vi "Channel Interface.vi"(8 "error in (no error)":errorcluster, 11 "Node Ptr":T1 format="%.0x") -> (0 "error out":errorcluster)   [LabVIEW 2020, in "SLSC EDS System Explorer.lvlib"]
uses:
  SLSC EDS System Explorer.lvlib
  <vilib>/NI VeriStand/Custom Device API/Custom Device Item Ref.ctl
  <vilib>/NI VeriStand/Custom Device API/Custom Device Channel Type.ctl
  <vilib>/NI VeriStand/Custom Device Tools/Custom Device Utility Library/Search Direction.ctl
  <vilib>/Utility/miscctls.llb/LVStringsAndValuesArrayTypeDef_U16.ctl
  Shared/Constants.vi
  <vilib>/NI VeriStand/Custom Device API/Get Item Property (String).vi
  <vilib>/NI VeriStand/Custom Device Tools/Custom Device Utility Library/NI VeriStand - Search for Item by GUID.vi
  <vilib>/NI VeriStand/Custom Device API/Custom Device API.lvlib
  Shared/SLSC EDS Shared.lvlib
  <vilib>/NI VeriStand/Custom Device Tools/Custom Device Utility Library/Custom Device Utility Library.lvlib
  SLSC CD API/SLSC CD Shared/SLSC CD Shared.lvlib
  SLSC UI API/SLSC Tree Control.lvlib
  SLSC CD API/SLSC CD System Explorer/SLSC CD System Explorer.lvlib
  <vilib>/NI VeriStand/Custom Device Tools/Custom Device Utility Library/NI VeriStand - Search for Item by Name.vi
panel:
  in  "Property tree":string[](tree)
  out "Physical Channel":string
  out "Property/Command Name":string
  out "Datatype":string
  in  "U8":u8 format="%.0x"
  in  "I8":i8
  in  "U32":u32 format="%.0x"
  in  "I32":i32
  in  "U64":u64 format="%.0x"
  in  "I64":i64
  in  "Ring":u16(ring)
  in  "DBL":dbl format="%#_16g"
  out "Documentation":string
  in  "Default Value":dbl
  out "Access":i32(ring) items=["None", "Read Only", "Write Only", "Read/Write"]
  out "SLSC Debugging Information":string
  in  "Header":cluster{"Section Name":string}={"Section Name"="Custom Device Item Settings"}
  out "Description":string
  out "Name":string
  # "Default Value"
  # "Channel Value"
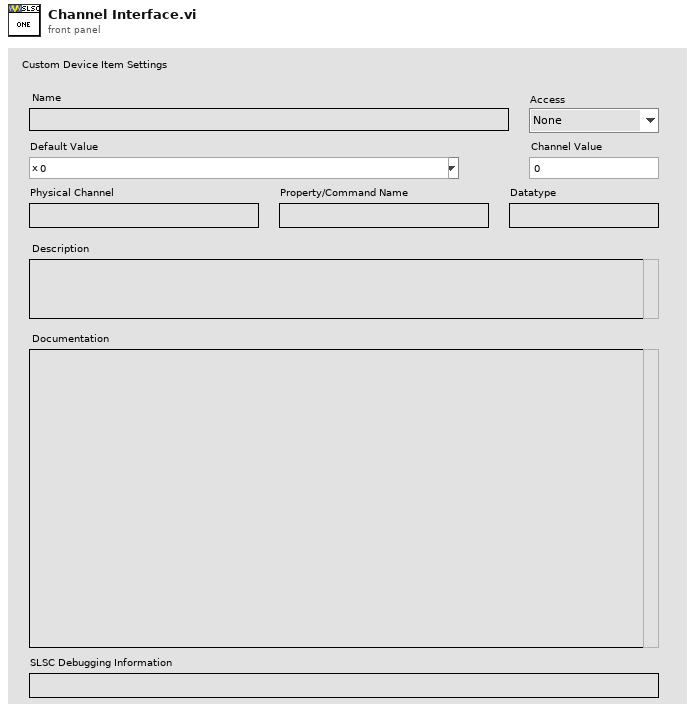
[diagram p1: front panel]
types:
  T1 = typedef "Custom Device API.lvlib/Custom Device Item Ref.ctl" = u64
  T2 = enum8{"Enabled", "Disabled", "Disabled and Grayed Out"}
  T3 = typedef "Custom Device Utility Library.lvlib/Search Direction.ctl" = enum16{"Down", "Up"}
  T4 = typedef "Custom Device API.lvlib/Custom Device Channel Type.ctl" = enum16{"Input", "Output"}
  T5 = typedef "LVStringsAndValuesArrayTypeDef_U16.ctl" = cluster{"String":string, "Value":u16}[]
  T6 = typedef "Custom Device API.lvlib/Custom Device Item Info.ctl" = cluster{"Name":string, "Is Channel":bool, "GUID":string, "Is Waveform":bool}
  T7 = typedef "EDSjsonStructure.ctl" = cluster{"vendorNum":u32, "vendorName":string, "vendorPrefix":string, "productNum":u32, "productName":string, "capsVersion":string, "capsSpecVersion":u32, "capsSpecOldestCompatibleVersion":u32, "enums":T8[], "properties":T9[], "commands":T10[], "scales":T11[], "physicalChannels":T12[], "registerMap":cluster{"registers":T13[]}}
  T8 = typedef "enum.ctl" = cluster{"name":string, "description-en":string, "values":cluster{"name":string, "description-en":string, "value":i32}[]}
  T9 = typedef "property.ctl" = cluster{"name":string, "description-en":string, "documentation-en":string, "dataType":string, "bitfield":string, "access":string, "scale":string, "value":variant, "min":variant, "max":variant, "default value":variant}
  T10 = typedef "command.ctl" = cluster{"name":string, "description-en":string, "documentation-en":string, "startBitfield":string, "waitTimeInMs":i32, "doneBitfield":string, "doneInterrupt":string, "doneTimeoutInMs":i32, "value":variant}
  T11 = typedef "scale.ctl" = cluster{"name":string, "description-en":string, "m":dbl, "b":dbl, "forwardCoeffs":dbl[], "reverseCoeffs":dbl[], "coercion":string, "table":cluster{"scaled":dbl, "unscaled":dbl}[]}
  T12 = typedef "physicalChannel.ctl" = cluster{"name":string, "description-en":string, "commands":T10[], "properties":T9[]}
  T13 = typedef "register.ctl" = cluster{"name":string, "description-en":string, "access":string, "address":u32, "size":u32, "bitfields":cluster{"name":string, "description-en":string, "offset":u32, "size":u32, "signed":bool, "strobe":bool}[]}
  T14 = typedef "Custom Device API.lvlib/Custom Device Channel.ctl" = cluster{"Type":T4, "Units":string, "Default Value":dbl, "Faultable":bool, "Scalable":bool}
  T15 = cluster{"Left Cell String":string, "Child Text":string[], "Child Tag":string, "Item Indent":i32, "Child Only?":bool, "Glyph Index":i32}[]
  T16 = cluster{"Left Cell String":string, "Child Text":string[], "Child Tag":string, "Item Indent":i32, "Child Only?":bool, "Glyph Index":i32}
  T17 = cluster{"name":string, "description-en":string, "value":i32}[]
  T18 = typedef "Custom Device API.lvlib/Custom Device Commands.ctl" = enum16{"Default", "Item renamed", "Shutdown", "Dynamic button pressed"}
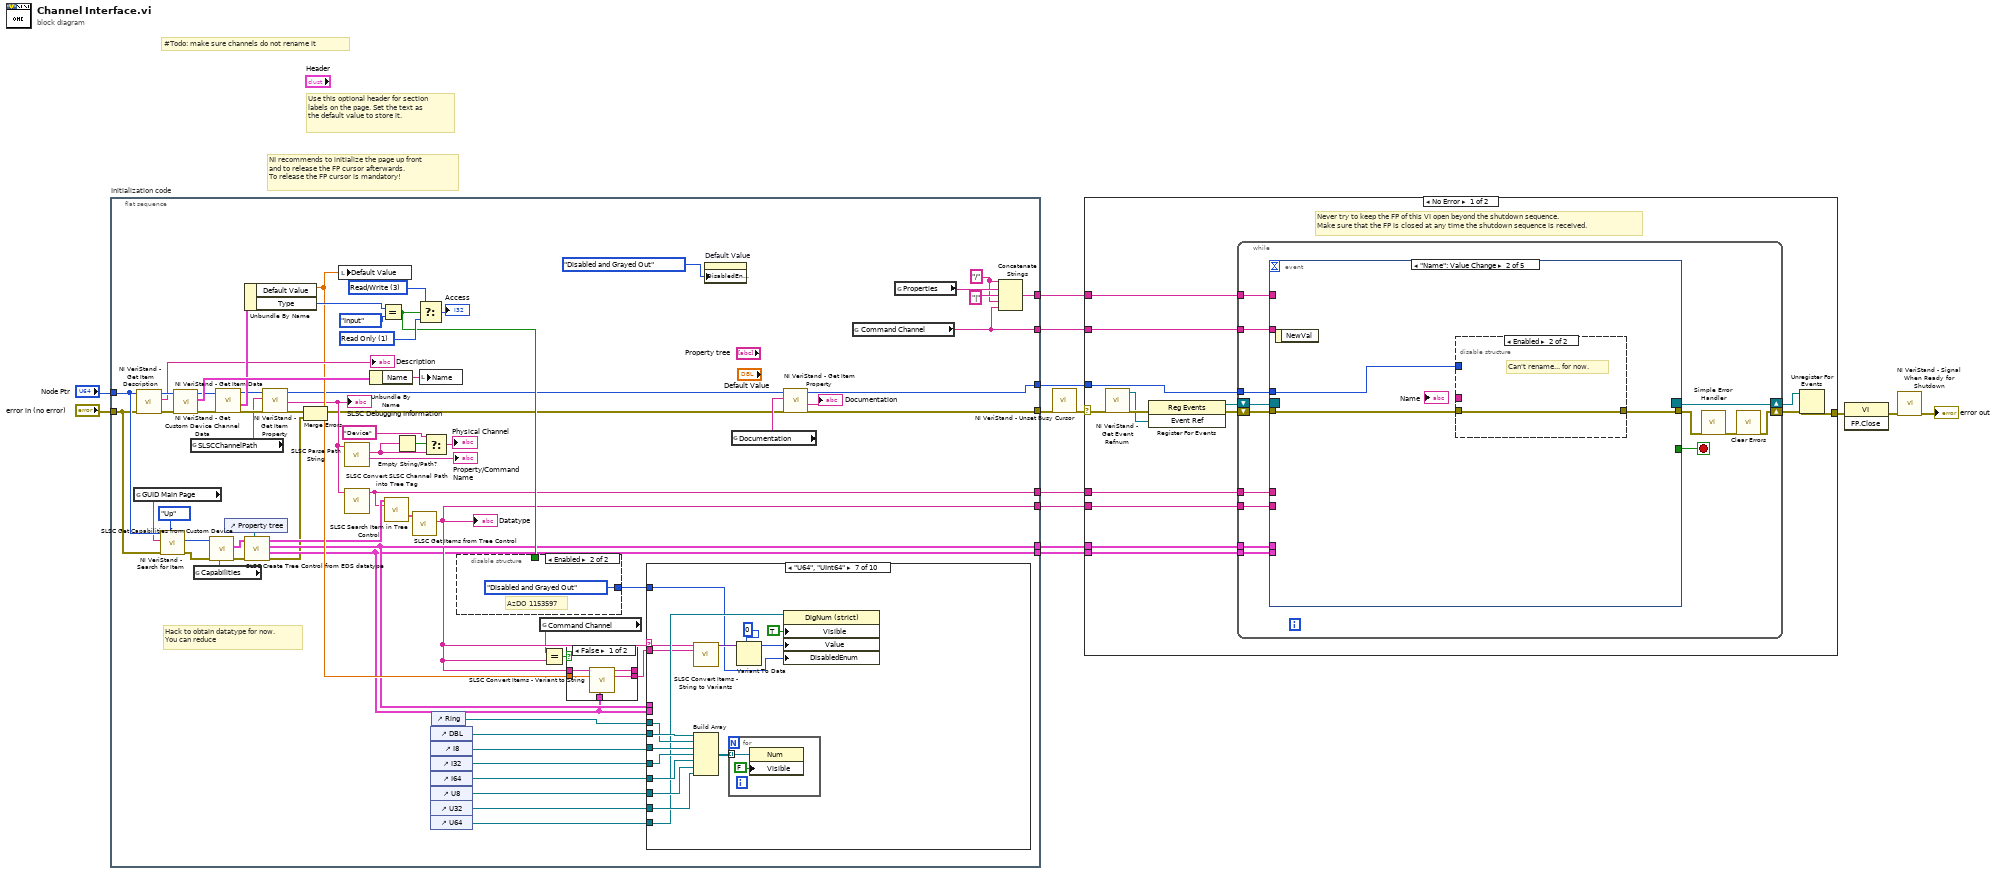
[diagram p0: block diagram]
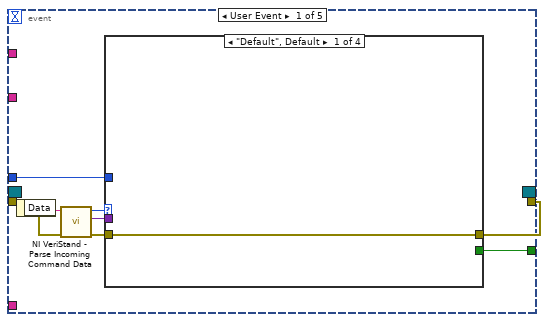
[diagram p2: hidden frame]
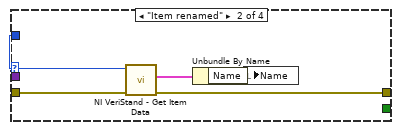
[diagram p3: hidden frame]
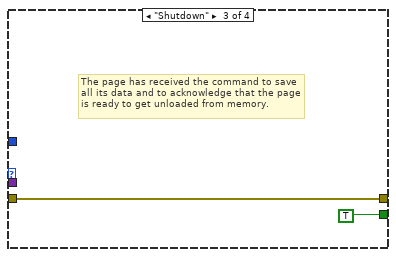
[diagram p4: hidden frame]
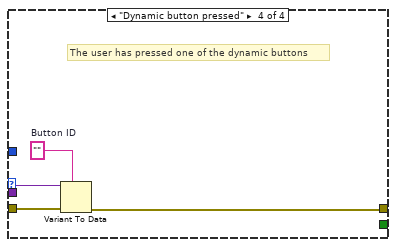
[diagram p5: hidden frame]
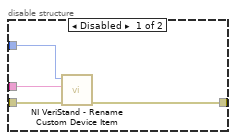
[diagram p6: hidden frame]
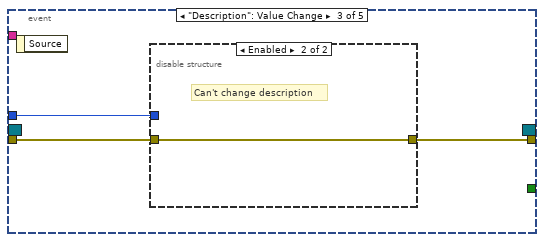
[diagram p7: hidden frame]
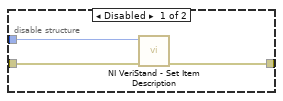
[diagram p8: hidden frame]
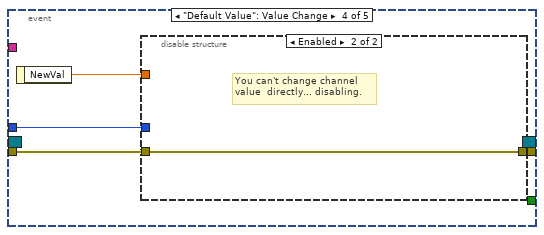
[diagram p9: hidden frame]
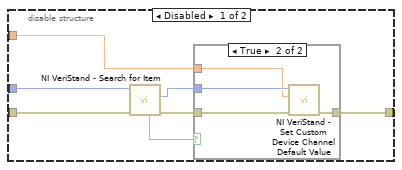
[diagram p10: hidden frame]
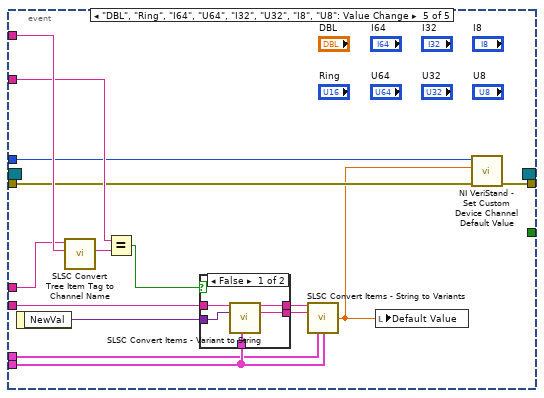
[diagram p12: hidden frame]
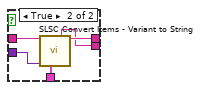
[diagram p13: hidden frame]
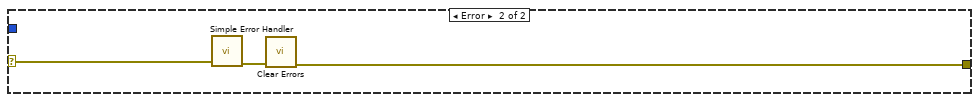
[diagram p14: hidden frame]
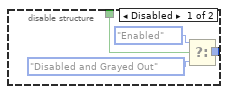
[diagram p15: hidden frame]
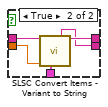
[diagram p16: hidden frame]
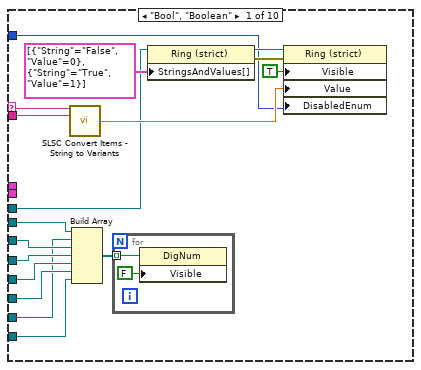
[diagram p17: hidden frame]
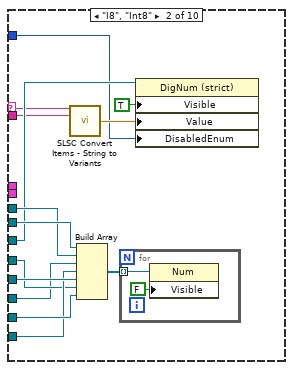
[diagram p18: hidden frame]
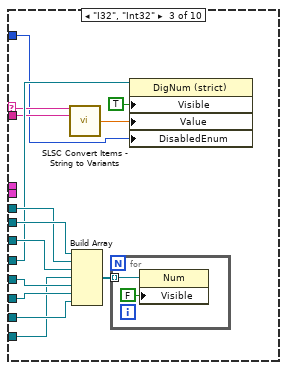
[diagram p19: hidden frame]
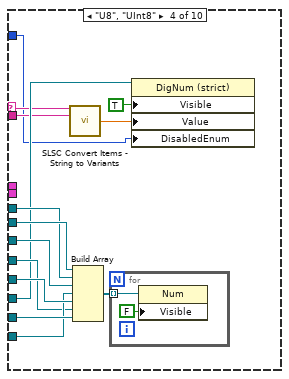
[diagram p20: hidden frame]
diagram:
  # "#Todo: make sure channels do not rename it"
  # "Use this optional header for section labels on the page. Set the text as the default value to store it."
  # "NI recommends to initialize the page up front\nand to release the FP cursor afterwards.\nTo release the FP cursor is mandatory!"
  n1 = flat-sequence "Initialization code" {
    tunnel: "error in (no error)" -> [w27]
    tunnel: "Node Ptr" -> [w52]
    tunnel: [w64] -> w10
    tunnel: [w22] -> w7
    tunnel: [w56] -> w6
    tunnel: [w48] -> w5
    tunnel: [w29] -> w4
    tunnel: [w35] -> w3
    tunnel: [w30] -> w2
    tunnel: [w31] -> w1
    frame #0 {
      w57 = "/" ("string")
      w77 = 1 items=["None", "Read Only", "Write Only", "Read/Write"] ("Access")
      w76 = 3 items=["None", "Read Only", "Write Only", "Read/Write"] ("Access")
      # "Hack to obtain datatype for now.\nYou can reduce"
      n2 = global read "Constants.vi" "GUID Main Page"() -> (w51:string)
      n3 = call <vilib>:"NI VeriStand - Get Item Description.vi"("error in (no error)"=w27, "Item Ref in"=w52) -> ("error out"=w79:errorcluster, "Description"=→"Description":string, "Item Ref out"=w80:T1)  [unwired: 7 out]
      n4 = call-poly <vilib>:"NI VeriStand - Search for Item.vi"("Direction (Down)"=Search_Direction."Up", "error in"=w27, "Item GUID"=w51, "Section Ref in"=w52) -> ("error out"=w28:errorcluster, "Item Ref"=w53:T1)  [unwired: 4 in, 2 out]
      n5 = call <vilib>:"NI VeriStand - Get Item Data.vi"("error in (no error)"=w79, "Item Ref in"=w80) -> ("error out"=w69:errorcluster, "Item Info"=w78:T6, "Item Ref out"=w70:T1)  [unwired: 7 out]
      n6 = global read "Constants.vi" "SLSCChannelPath"() -> (w68:string)
      n7 = global read "Constants.vi" "Capabilities"() -> (w60:string)
      n8 = call "SLSC Get Capabilities from Custom Device.vi"("Property Name"=w60, "error in (no error)"=w28, "Device Item Ref in"=w53) -> ("error out"=w24:errorcluster, "data"=w36:T7)  [unwired: 3 in, 4 out]
      n9 = call <vilib>:"NI VeriStand - Get Custom Device Channel Data.vi"("error in (no error)"=w69, "Channel Ref in"=w70) -> ("error out"=w72:errorcluster, "Channel"=w71:T14, "Channel Ref out"=w66:T1)  [unwired: 4 in, 3 out]
      n10 = control-ref of="Property tree"() -> (w37:refnum<vi>)
      n11 = Unbundle By Name(w71) -> ("Default Value"=w49:dbl, "Type"=w73:T4)
      n12 = call "SLSC Create Tree Control from EDS datatype.vi"("Property Tree"=w37, "error in (no error)"=w24, "SLSC EDS module"=w36) -> ("error out"=w18:errorcluster, "Enum Strings"=w29:cluster{"name":string, string}[], "Enums"=w35:T8[], "SLSC Output Tree"=w34:T15)  [unwired: 5 in]
      n13 = call-poly <vilib>:"NI VeriStand - Get Item Property.vi"("error in (no error)"=w72, "Property Name"=w68, "Item Ref in"=w66) -> ("error out"=w20:errorcluster, "Value"=w33:string, "Item Ref out"=w21:T1)  [unwired: 5 in, 1 out]
      "SLSC Debugging Information" <- w33
      n14 = Merge Errors(w20, w18) -> (w19:errorcluster)
      n15 = local write "Default Value"(w49) -> ()
      n16 = call "SLSC Parse Path String.vi"("SLSC Channel Path"=w33) -> ("Property or Command"=→"Property/Command Name":string, "Physical Channel"=w39:string)  [unwired: 7 in, 2 out]
      n17 = call "SLSC Convert SLSC Channel Path into Tree Tag.vi"("SLSC Channel Path"=w33) -> ("Tree Item Channel"=w31:string)  [unwired: 9 in, 1 out]
      n18 = Unbundle By Name(w78) -> ("Name"=w61:string)
      n19 = Equal?(x=w73, y=Custom_Device_Channel_Type."Input") -> (x = y?=w62:bool)
      n20 = call "SLSC Search Item in Tree Control.vi"("SLSC Output Tree"=w34, "Item Tag"=w31) -> ("Item"=w32:T16)  [unwired: 10 in, 3 out]
      n21 = Empty String/Path?(string/path=w39) -> (empty?=w41:bool)
      n22 = call "SLSC Get Items from Tree Control.vi"("Item"=w32) -> ("Datatype"=w30:string)  [unwired: 6 in, 4 out]
      "Datatype" <- w30
      n23 = Select(t=w76, s=w62, f=w77) -> (s? t:f=→"Access":i32)
      n24 = local write "Name"(w61) -> ()
      n25 = Select(t="Device", s=w41, f=w39) -> (s? t:f=→"Physical Channel":string)
      n26 = control-ref of="DBL"() -> (w43:refnum<vi>)
      n27 = control-ref of="I8"() -> (w55:refnum<vi>)
      n28 = control-ref of="I32"() -> (w54:refnum<vi>)
      n29 = control-ref of="I64"() -> (w44:refnum<vi>)
      n30 = control-ref of="U8"() -> (w47:refnum<vi>)
      n31 = control-ref of="U32"() -> (w46:refnum<vi>)
      n32 = control-ref of="U64"() -> (w45:refnum<vi>)
      n33 = control-ref of="Ring"() -> (w16:refnum<vi>)
      n34 = disable-structure shown="Enabled" {
        disable-tunnel: w62 -> [w84 _]
        disable-tunnel: [w81 T2."Disabled and Grayed Out" ("Disabled")] -> w15
        frame Disabled {
          n35 = Select(t=T2."Enabled" ("Disabled"), s=w84, f=T2."Disabled and Grayed Out" ("Disabled")) -> (s? t:f=w81:T2)
        }
        frame Enabled {
          # "AzDO 1153597"
        }
      }
      n36 = global read "Constants.vi" "Command Channel"() -> (w23:string)
      n37 = Equal?(x=w23, y=w30) -> (x = y?=w26:bool)
      n38 = case shown="False" w26 {
        tunnel: w49 -> [w90 w92]
        tunnel: [w89 w91] -> w25
        tunnel: [w88 w95] -> _
        tunnel: w30 -> [w87 w94]
        tunnel: w29 -> [w86 w93]
        frame False {
          n39 = call "SLSC Convert Items - Variant to String.vi"("Datatype"=w87, "value"=w90, "Enum string"=w86) -> ("Output data type"=w88:string, "string data value"=w89:string)  [unwired: 6 in, 5 out]
        }
        frame True {
          n40 = call "SLSC Convert Items - Variant to String.vi"("Datatype"=w94, "reset value"=w92, "Enum string"=w93) -> ("string data reset value"=w91:string, "Output data type"=w95:string)  [unwired: 6 in, 5 out]
        }
      }
      n41 = case shown="\"U64\", \"UInt64\"" w30 {
        selector: w30 -> [w102 w119 w135 w151 w167 w181 w201 w219 w236 w267]
        tunnel: w16 -> [w98 w127 w143 w159 w174 w193 w211 w228 w232 w259]
        tunnel: w46 -> [w105 w124 w138 w155 w176 w188 w205 w222 w241 w271]
        tunnel: w43 -> [w112 w128 w144 w160 w175 w194 w212 w221 w246 w276]
        tunnel: w55 -> [w111 w120 w142 w158 w173 w192 w210 w227 w245 w275]
        tunnel: w54 -> [w110 w122 w136 w153 w172 w191 w209 w226 w244 w274]
        tunnel: w44 -> [w109 w126 w141 w157 w171 w186 w208 w225 w243 w273]
        tunnel: w47 -> [w108 w121 w140 w152 w170 w190 w207 w224 w242 w272]
        tunnel: w45 -> [w107 w123 w137 w154 w169 w187 w204 w220 w240 w270]
        tunnel: w35 -> [_ _ _ _ _ _ _ _ w247 _]
        tunnel: w25 -> [w101 w118 w134 w150 w166 w180 w200 w218 w238 w268]
        tunnel: w29 -> [_ _ _ _ _ _ _ _ w237 _]
        tunnel: w15 -> [w96 w115 w131 w147 w163 w179 w197 w215 w231 _]
        frame "Bool", "Boolean" {
          n42 = call "SLSC Convert Items - String to Variants.vi"("Datatype"=w102, "Value"=w101) -> ("Value (DBL)"=w100:dbl)  [unwired: 10 in, 3 out]
          n43 = Build Array(w112, w105, w111, w110, w109, w108, w107) -> (w106:refnum<vi>[])
          n44 = for {
            tunnel: w106 -> [w114] mode=indexing
            n45 = property class="DigNum"(reference=w114, "Visible"=FALSE) -> ()  [unwired: 1 in, 2 out]
          }
          n46 = property on="Property Node" class="Ring (strict)"(reference=w98, "StringsAndValues[]"=T5 [{"String"="False", "Value"=0}, {"String"="True", "Value"=1}] ("Strings And Values []")) -> (reference out=w97:refnum<vi>, error out=w103:errorcluster)  [unwired: 1 in]
          n47 = property class="Ring (strict)"(reference=w97, error in=w103, "Visible"=TRUE, "Value"=w100, "DisabledEnum"=w96) -> ()  [unwired: 2 out]
        }
        frame "I8", "Int8" {
          n48 = call "SLSC Convert Items - String to Variants.vi"("Datatype"=w119, "Value"=w118) -> ("Value (DBL)"=w117:dbl)  [unwired: 10 in, 3 out]
          n49 = Build Array(w128, w127, w121, w123, w126, w122, w124) -> (w125:refnum<vi>[])
          n50 = for {
            tunnel: w125 -> [w130] mode=indexing
            n51 = property class="Num"(reference=w130, "Visible"=FALSE) -> ()  [unwired: 1 in, 2 out]
          }
          n52 = property class="DigNum (strict)"(reference=w120, "Visible"=TRUE, "Value"=w117, "DisabledEnum"=w115) -> ()  [unwired: 1 in, 2 out]
        }
        frame "I32", "Int32" {
          n53 = call "SLSC Convert Items - String to Variants.vi"("Datatype"=w135, "Value"=w134) -> ("Value (DBL)"=w133:dbl)  [unwired: 10 in, 3 out]
          n54 = Build Array(w144, w143, w142, w137, w141, w140, w138) -> (w139:refnum<vi>[])
          n55 = for {
            tunnel: w139 -> [w146] mode=indexing
            n56 = property class="Num"(reference=w146, "Visible"=FALSE) -> ()  [unwired: 1 in, 2 out]
          }
          n57 = property class="DigNum (strict)"(reference=w136, "Visible"=TRUE, "Value"=w133, "DisabledEnum"=w131) -> ()  [unwired: 1 in, 2 out]
        }
        frame "U8", "UInt8" {
          n58 = call "SLSC Convert Items - String to Variants.vi"("Datatype"=w151, "Value"=w150) -> ("Value (DBL)"=w149:dbl)  [unwired: 10 in, 3 out]
          n59 = Build Array(w160, w159, w158, w154, w157, w153, w155) -> (w156:refnum<vi>[])
          n60 = for {
            tunnel: w156 -> [w162] mode=indexing
            n61 = property class="Num"(reference=w162, "Visible"=FALSE) -> ()  [unwired: 1 in, 2 out]
          }
          n62 = property class="DigNum (strict)"(reference=w152, "Visible"=TRUE, "Value"=w149, "DisabledEnum"=w147) -> ()  [unwired: 1 in, 2 out]
        }
        frame "U32", "UInt32" {
          n63 = Build Array(w175, w174, w173, w172, w171, w170, w169) -> (w168:refnum<vi>[])
          n64 = call "SLSC Convert Items - String to Variants.vi"("Datatype"=w167, "Value"=w166) -> ("Value (DBL)"=w165:dbl)  [unwired: 10 in, 3 out]
          n65 = for {
            tunnel: w168 -> [w178] mode=indexing
            n66 = property class="Num"(reference=w178, "Visible"=FALSE) -> ()  [unwired: 1 in, 2 out]
          }
          n67 = property class="DigNum (strict)"(reference=w176, "Visible"=TRUE, "Value"=w165, "DisabledEnum"=w163) -> ()  [unwired: 1 in, 2 out]
        }
        frame "I64", "Int64" {
          n68 = call "SLSC Convert Items - String to Variants.vi"("Datatype"=w181, "Value"=w180) -> ("Value"=w185:variant)  [unwired: 10 in, 3 out]
          n69 = Build Array(w194, w193, w192, w191, w187, w190, w188) -> (w189:refnum<vi>[])
          n70 = for {
            tunnel: w189 -> [w196] mode=indexing
            n71 = property class="Num"(reference=w196, "Visible"=FALSE) -> ()  [unwired: 1 in, 2 out]
          }
          n72 = Variant To Data(type=i64 0, Variant=w185) -> (data=w183:i64)  [unwired: 1 in, 1 out]
          n73 = property class="DigNum (strict)"(reference=w186, "Visible"=TRUE, "Value"=w183, "DisabledEnum"=w179) -> ()  [unwired: 1 in, 2 out]
        }
        frame "U64", "UInt64" {
          n74 = call "SLSC Convert Items - String to Variants.vi"("Datatype"=w201, "Value"=w200) -> ("Value"=w199:variant)  [unwired: 10 in, 3 out]
          n75 = Build Array(w212, w211, w210, w209, w208, w207, w205) -> (w206:refnum<vi>[])
          n76 = for {
            tunnel: w206 -> [w214] mode=indexing
            n77 = property class="Num"(reference=w214, "Visible"=FALSE) -> ()  [unwired: 1 in, 2 out]
          }
          n78 = Variant To Data(type=u64 0, Variant=w199) -> (data=w202:u64)  [unwired: 1 in, 1 out]
          n79 = property class="DigNum (strict)"(reference=w204, "Visible"=TRUE, "Value"=w202, "DisabledEnum"=w197) -> ()  [unwired: 1 in, 2 out]
        }
        frame "DBL", "Double" {
          n80 = call "SLSC Convert Items - String to Variants.vi"("Datatype"=w219, "Value"=w218) -> ("Value (DBL)"=w217:dbl)  [unwired: 10 in, 3 out]
          n81 = Build Array(w220, w228, w227, w226, w225, w224, w222) -> (w223:refnum<vi>[])
          n82 = for {
            tunnel: w223 -> [w230] mode=indexing
            n83 = property class="Num"(reference=w230, "Visible"=FALSE) -> ()  [unwired: 1 in, 2 out]
          }
          n84 = property class="DigNum (strict)"(reference=w221, "Visible"=TRUE, "Value"=w217, "DisabledEnum"=w215) -> ()  [unwired: 1 in, 2 out]
        }
        frame Default {
          n85 = Build Array(w246, w245, w244, w243, w242, w241, w240) -> (w239:refnum<vi>[])
          n86 = call "SLSC Search and Convert ENUM Value by Name.vi"("Enum Strings"=w237, "enums"=w247, "Value"=w238, "Datatype Name"=w236) -> ("Enum"=w234:T8, "Datatype found?"=w233:bool, "Value"=w235:i32)  [unwired: 5 in]
          n87 = for {
            tunnel: w239 -> [w249] mode=indexing
            n88 = property class="DigNum"(reference=w249, "Visible"=FALSE) -> ()  [unwired: 1 in, 2 out]
          }
          n89 = case shown="True" w233 {
            tunnel: w234 -> [_ w253]
            tunnel: w232 -> [_ w250]
            frame False {
              # "Datatype not found: hide all controls"
            }
            frame True {
              # "Show Ring control for custom datatype"
              n90 = Unbundle By Name(w253) -> ("values"=w252:T17)
              n91 = for {
                tunnel: w252 -> [w257] mode=indexing
                tunnel: [w254] -> w251 mode=indexing
                n92 = Unbundle(w257) -> ("name"=w256:string, "value"=w255:i32)  [unwired: 1 out]
                n93 = Bundle("name"=w256, "value"=w255) -> (w254:cluster{"name":string, "value":i32})  [unwired: 1 in]
              }
              n94 = property on="Property Node" class="Ring (strict)"(reference=w250, "StringsAndValues[]"=w251) -> ()  [unwired: 1 in, 2 out]
            }
          }
          n95 = property class="Ring (strict)"(reference=w232, "Visible"=w233, "Value"=w235, "DisabledEnum"=w231) -> ()  [unwired: 1 in, 2 out]
        }
        frame "Command" {
          n96 = Build Array(w276, w275, w274, w273, w272, w271, w270) -> (w269:refnum<vi>[])
          n97 = call "SLSC Command Enum Constant.vi"("Option on Reset?"=FALSE) -> ("Array"=w264:T8[])  [unwired: 10 in, 4 out]
          n98 = for {
            tunnel: w269 -> [w282] mode=indexing
            n99 = property class="DigNum"(reference=w282, "Visible"=FALSE) -> ()  [unwired: 1 in, 2 out]
          }
          n100 = call "SLSC Search and Convert ENUM Value by Name.vi"("enums"=w264, "Value"=w268, "Datatype Name"=w267) -> ("Enum"=w265:T8, "Value"=w266:i32)  [unwired: 6 in, 1 out]
          n101 = Unbundle By Name(w265) -> ("values"=w262:T17)
          n102 = for {
            tunnel: w262 -> [w280] mode=indexing
            tunnel: [w277] -> w261 mode=indexing
            n103 = Unbundle(w280) -> ("name"=w279:string, "value"=w278:i32)  [unwired: 1 out]
            n104 = Bundle("name"=w279, "value"=w278) -> (w277:cluster{"name":string, "value":i32})  [unwired: 1 in]
          }
          n105 = property class="Ring (strict)"(reference=w259, "Visible"=TRUE, "Value"=w266, "DisabledEnum"=T2."Disabled and Grayed Out" ("Disabled")) -> ()  [unwired: 1 in, 2 out]
          n106 = property on="Property Node" class="Ring (strict)"(reference=w259, "StringsAndValues[]"=w261) -> ()  [unwired: 1 in, 2 out]
        }
      }
      n107 = property on="Default Value" class="DigNum (strict)"("DisabledEnum"=T2."Disabled and Grayed Out" ("Disabled")) -> ()  [unwired: 2 in, 2 out]
      n108 = global read "Constants.vi" "Documentation"() -> (w67:string)
      n109 = call-poly <vilib>:"NI VeriStand - Get Item Property.vi"("error in (no error)"=w19, "Property Name"=w67, "Item Ref in"=w21) -> ("error out"=w64:errorcluster, "Value"=→"Documentation":string, "Item Ref out"=w22:T1)  [unwired: 5 in, 1 out]
      n110 = global read "Constants.vi" "Command Channel"() -> (w48:string)
      n111 = global read "Constants.vi" "Properties"() -> (w58:string)
      n112 = Concatenate Strings(w57, w58, "|" ("string"), w57, w48) -> (w56:string)
    }
  }
  n113 = call <vilib>:"NI VeriStand - Unset Busy Cursor.vi"("error in (no error)"=w10) -> ("error out"=w9:errorcluster)  [unwired: 10 out]
  n114 = case shown="No Error" w9 {
    selector: w9 -> [w289 w389]
    tunnel: [w294 w390] -> w14
    tunnel: w7 -> [w290 _]
    tunnel: w1 -> [w288 _]
    tunnel: w6 -> [w287 _]
    tunnel: w5 -> [w286 _]
    tunnel: w4 -> [w285 _]
    tunnel: w3 -> [w284 _]
    tunnel: w2 -> [w283 _]
    frame No Error {
      # "Never try to keep the FP of this VI open beyond the shutdown sequence.\nMake sure that the FP is closed at any time the shutdown sequence is received."
      n115 = call <vilib>:"NI VeriStand - Get Event Refnum.vi"("error in (no error)"=w289) -> ("error out"=w297:errorcluster, "Event Ref"=w293:refnum<user-event>)  [unwired: 9 out]
      n116 = register-events(error in=w297, w293) -> (reference out=w291:refnum<event-registration>, error out=w292:errorcluster)  [unwired: 1 in]
      n117 = while {
        tunnel: w290 -> [w307]
        shift-right: [w305] -> w295
        shift-left: w292 -> [w310]
        shift-right: [w311] -> w296
        shift-left: w291 -> [w309]
        tunnel: w288 -> [w304]
        tunnel: w287 -> [w303]
        tunnel: w286 -> [w302]
        tunnel: w285 -> [w301]
        tunnel: w284 -> [w300]
        tunnel: w283 -> [w299]
        stop <- w308 stop-if-true
        n118 = event shown="[1] \"Name\": Value Change" {
          selector: w309 -> [_ _ _ _ _]
          dyn-events: [_ _ _ _ _] -> w311
          timeout: _ -> [_ _ _ _ _]
          tunnel: w310 -> [w319 w334 w341 w348 w369]
          tunnel: [w315 _ _ _ _] -> w308
          tunnel: [w314 w333 w340 w347 w371] -> w298
          tunnel: w307 -> [w313 w332 w342 w350 w370]
          tunnel: w304 -> [_ _ _ _ w364]
          tunnel: w303 -> [_ _ _ _ w374]
          tunnel: w302 -> [_ _ _ _ w373]
          tunnel: w301 -> [_ _ _ _ w367]
          tunnel: w300 -> [_ _ _ _ w366]
          tunnel: w299 -> [_ _ _ _ w365]
          event User Event {
            n119 = event-data() -> ("Data"=w318:string)  [unwired: 1 out]
            n120 = call <vilib>:"NI VeriStand - Parse Incoming Command Data.vi"("error in (no error)"=w319, "Incoming data"=w318) -> ("error out"=w317:errorcluster, "Outgoing data"=w312:variant, "Action"=w316:T18)  [unwired: 7 out]
            n121 = case shown="\"Default\", Default" w316 {
              tunnel: w317 -> [w320 w325 w326 w331]
              tunnel: [_ _ TRUE _] -> w315
              tunnel: [w320 w322 w326 w328] -> w314
              tunnel: w313 -> [_ w324 _ _]
              tunnel: w312 -> [_ _ _ w330]
              frame "Default", Default {
              }
              frame "Item renamed" {
                n122 = call <vilib>:"NI VeriStand - Get Item Data.vi"("error in (no error)"=w325, "Item Ref in"=w324) -> ("error out"=w322:errorcluster, "Item Info"=w323:T6)  [unwired: 8 out]
                n123 = Unbundle By Name(w323) -> ("Name"=w321:string)
                n124 = local write "Name"(w321) -> ()
              }
              frame "Shutdown" {
                # "The page has received the command to save all its data and to acknowledge that the page is ready to get unloaded from memory."
              }
              frame "Dynamic button pressed" {
                w329 = ""  # Button ID
                # "The user has pressed one of the dynamic buttons"
                n125 = Variant To Data(error in=w331, type=w329, Variant=w330) -> (error out=w328:errorcluster)  [unwired: 1 out]
              }
            }
          }
          event "Name": Value Change {
            n126 = event-data() -> ()  [unwired: 2 out]
            n127 = disable-structure shown="Enabled" {
              disable-tunnel: w334 -> [w338 w339]
              disable-tunnel: [w337 w339] -> w333
              disable-tunnel: w332 -> [w336 _]
              disable-tunnel: _ -> [w335 _]
              frame Disabled {
                n128 = call <vilib>:"NI VeriStand - Rename Custom Device Item.vi"("error in (no error)"=w338, "New Name"=w335, "Item Ref in"=w336) -> ("error out"=w337:errorcluster)  [unwired: 1 in, 7 out]
              }
              frame Enabled {
                # "Can't rename... for now."
              }
            }
          }
          event "Description": Value Change {
            n129 = event-data() -> ()  [unwired: 2 out]
            n130 = disable-structure shown="Enabled" {
              disable-tunnel: w342 -> [w345 _]
              disable-tunnel: w341 -> [w344 w346]
              disable-tunnel: [w343 w346] -> w340
              frame Disabled {
                n131 = call <vilib>:"NI VeriStand - Set Item Description.vi"("error in (no error)"=w344, "Item Ref in"=w345) -> ("error out"=w343:errorcluster)  [unwired: 1 in, 8 out]
              }
              frame Enabled {
                # "Can't change description"
              }
            }
          }
          event "Default Value": Value Change {
            n132 = event-data() -> ("NewVal"=w349:dbl)  [unwired: 1 out]
            n133 = disable-structure shown="Enabled" {
              disable-tunnel: w350 -> [w357 _]
              disable-tunnel: w349 -> [w355 _]
              disable-tunnel: w348 -> [w354 w363]
              disable-tunnel: [w352 w363] -> w347
              frame Disabled {
                n134 = call-poly <vilib>:"NI VeriStand - Search for Item.vi"("error in"=w354, "Section Ref in"=w357) -> ("error out"=w353:errorcluster, "Item Ref"=w356:T1, "Found"=w351:bool)  [unwired: 6 in, 1 out]
                n135 = case shown="True" w351 {
                  tunnel: w356 -> [_ w362]
                  tunnel: w355 -> [_ w361]
                  tunnel: w353 -> [w358 w360]
                  tunnel: [w358 w359] -> w352
                  frame False {
                  }
                  frame True {
                    n136 = call <vilib>:"NI VeriStand - Set Custom Device Channel Default Value.vi"("error in (no error)"=w360, "Default Value"=w361, "Channel Ref in"=w362) -> ("error out"=w359:errorcluster)  [unwired: 7 in, 1 out]
                  }
                }
              }
              frame Enabled {
                # "You can't change channel \nvalue  directly... disabling."
              }
            }
          }
          event "DBL", "Ring", "I64", "U64", "I32", "U32", "I8", "U8": Value Change {
            n137 = event-data() -> ("NewVal"=w378:variant)  [unwired: 1 out]
            n138 = call "SLSC Convert Tree Item Tag to Channel Name.vi"("Type of Item"=w374, "Item String"=w364) -> ("Type of Item"=w375:string)  [unwired: 7 in, 2 out]
            n139 = Equal?(x=w373, y=w375) -> (x = y?=w372:bool)
            n140 = case shown="False" w372 {
              tunnel: w378 -> [w383 w385]
              tunnel: [w382 w384] -> w376
              tunnel: [w381 w388] -> w377
              tunnel: w365 -> [w380 w387]
              tunnel: w367 -> [w379 w386]
              frame False {
                n141 = call "SLSC Convert Items - Variant to String.vi"("Datatype"=w380, "value"=w383, "Enum string"=w379) -> ("Output data type"=w381:string, "string data value"=w382:string)  [unwired: 6 in, 5 out]
              }
              frame True {
                n142 = call "SLSC Convert Items - Variant to String.vi"("Datatype"=w387, "reset value"=w385, "Enum string"=w386) -> ("string data reset value"=w384:string, "Output data type"=w388:string)  [unwired: 6 in, 5 out]
              }
            }
            n143 = call "SLSC Convert Items - String to Variants.vi"("Datatype"=w377, "Value"=w376, "enums"=w366, "string enums"=w367) -> ("Value (DBL)"=w368:dbl)  [unwired: 8 in, 3 out]
            n144 = local write "Default Value"(w368) -> ()
            n145 = call <vilib>:"NI VeriStand - Set Custom Device Channel Default Value.vi"("error in (no error)"=w369, "Default Value"=w368, "Channel Ref in"=w370) -> ("error out"=w371:errorcluster)  [unwired: 7 in, 1 out]
          }
        }
        n146 = call <vilib>:"Simple Error Handler.vi"("error in (no error)"=w298) -> ("error out"=w306:errorcluster)  [unwired: 1 in, 7 out]
        n147 = call <vilib>:"Clear Errors.vi"("error in (no error)"=w306) -> ("error out"=w305:errorcluster)  [unwired: 1 in, 5 out]
      }
      n148 = Unregister For Events(event registration refnum=w296, error in=w295) -> (error out=w294:errorcluster)
    }
    frame Error {
      n149 = call <vilib>:"Simple Error Handler.vi"("error in (no error)"=w389) -> ("error out"=w391:errorcluster)  [unwired: 1 in, 7 out]
      n150 = call <vilib>:"Clear Errors.vi"("error in (no error)"=w391) -> ("error out"=w390:errorcluster)  [unwired: 1 in, 5 out]
    }
  }
  n151 = invoke class="VI" method="FP.Close"(error in=w14) -> (error out=w13:errorcluster)  [unwired: 2 in, 2 out]
  n152 = call <vilib>:"NI VeriStand - Signal When Ready for Shutdown.vi"("error in (no error)"=w13) -> ("error out"=→"error out":errorcluster)  [unwired: 10 out]
